vi "MQTT Packet - Receive.vi"(0 "mqtt ref in":T1, 7 "timeout (global)":i32=-1, 11 "error in":errorcluster) -> (3 "RAW data":string, 4 "mqtt ref out":T1, 6 "Fixed Header":T2, 8 "Remaining Data":u8[](array[numeric]), 10 "TimedOut":bool, 15 "error out":errorcluster)   [LabVIEW 2019, in "KoRE-MQTT.lvlib"]
doc: "Copyright (c) 2025 KoRElibs.com\nSPDX-License-Identifier: EUPL-1.2\n\nThis VI is licensed under the European Union Public License (EUPL) Version 1.2. You may use this VI unmodified in proprietary works. If you distribute a modified version of this file, the modified file must be released under the EUPL-1.2. Full license: https://joinup.ec.europa.eu/asset/eupl/eupl/1.2/"
uses:
  KoRE-MQTT.lvlib
  TypeDefs/MQTT Packet - Fixed Header.ctl
  TypeDefs/MQTT Packet - Type.ctl
  Public/TypeDefs/MQTT Client Session.ctl
  MQTT Data Stream - Decode Varint.vi
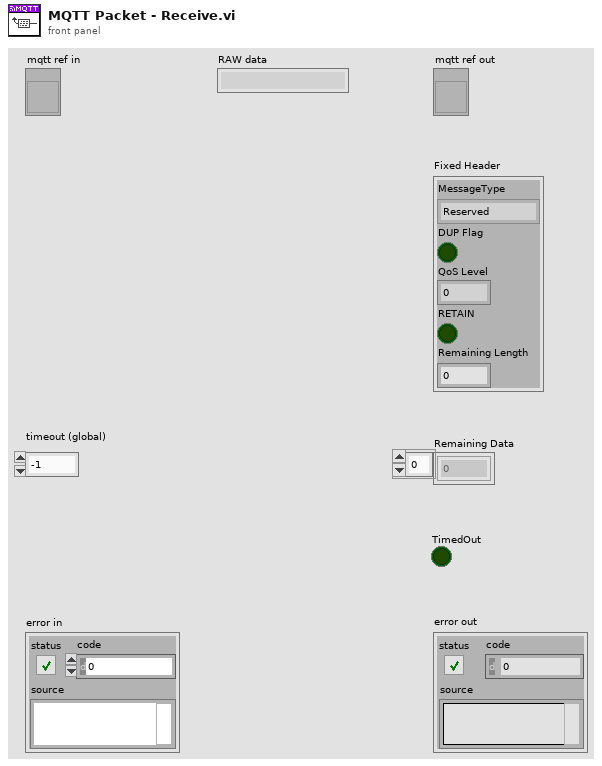
[diagram p1: front panel]
types:
  T1 = typedef "KoRE-MQTT.lvlib/MQTT Client Session.ctl" = refnum<vi>
  T2 = typedef "KoRE-MQTT.lvlib/MQTT Packet - Fixed Header.ctl" = cluster{"MessageType":T3, "DUP Flag":bool, "QoS Level":u8, "RETAIN":bool, "Remaining Length":u32}
  T3 = typedef "KoRE-MQTT.lvlib/MQTT Packet - Type.ctl" = enum32{"Reserved", "CONNECT", "CONNACK", "PUBLISH", "PUBACK", "PUBREC", "PUBREL", "PUBCOMP", "SUBSCRIBE", "SUBACK", "UNSUBSCRIBE", "UNSUBACK", "PINGREQ", "PINGRESP", "DISCONNECT", "AUTH"}
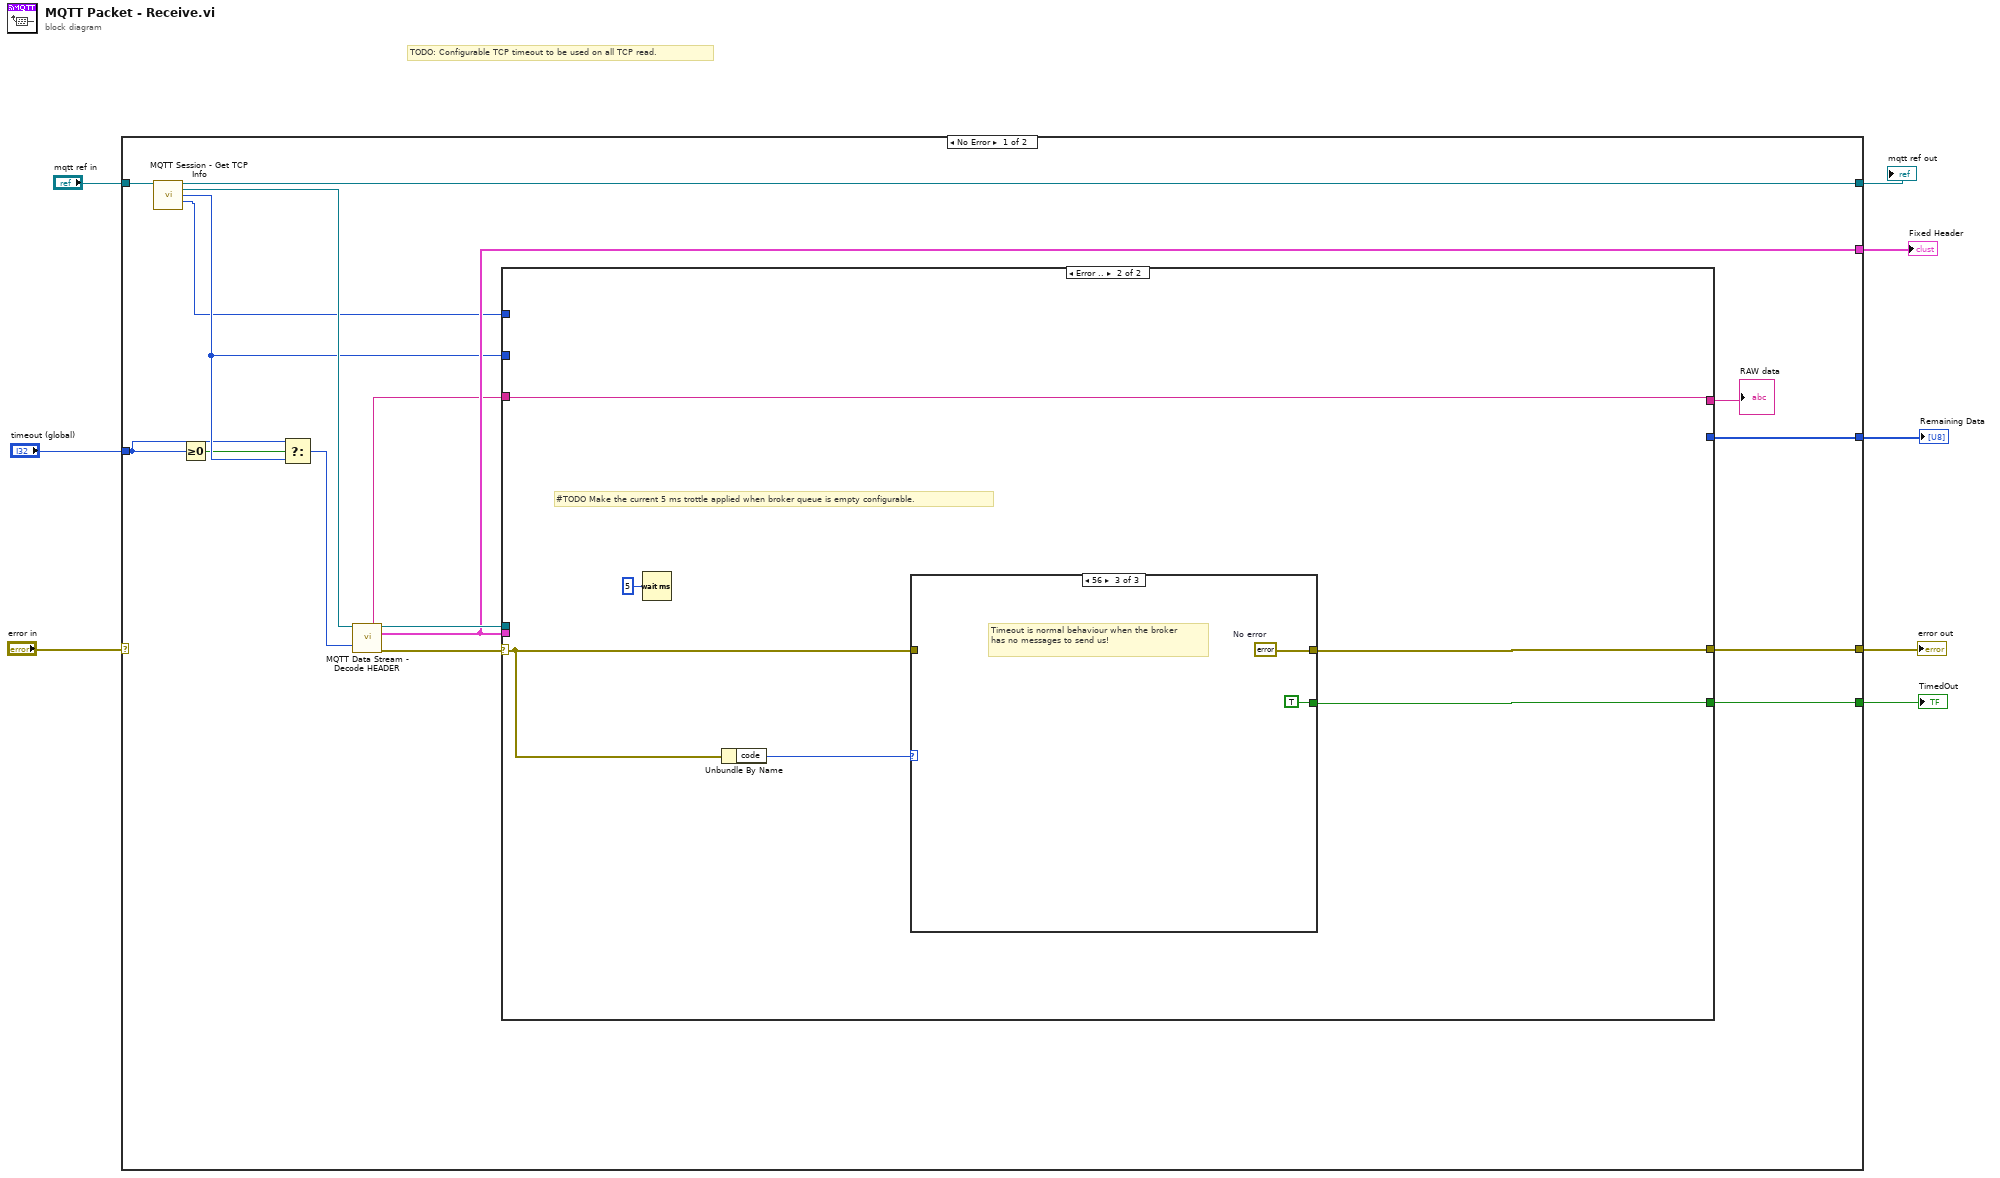
[diagram p0: block diagram]
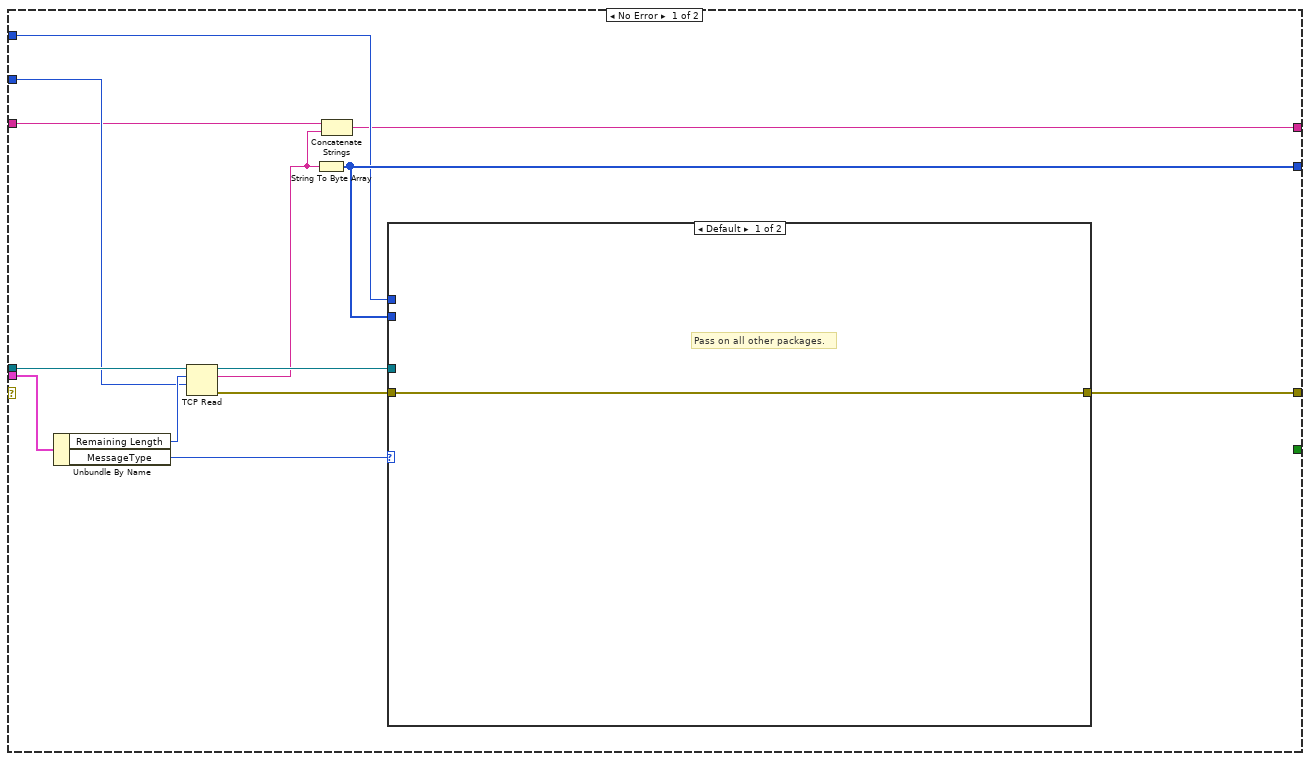
[diagram p2: hidden frame]
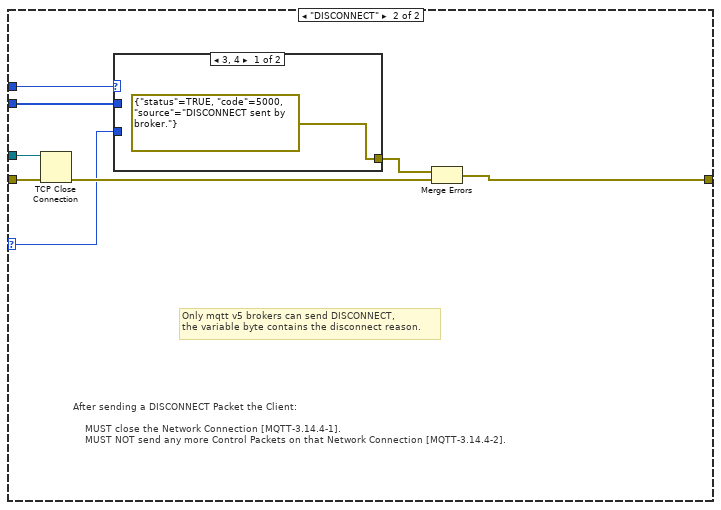
[diagram p3: hidden frame]
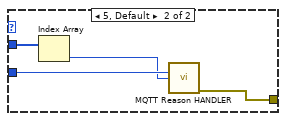
[diagram p4: hidden frame]
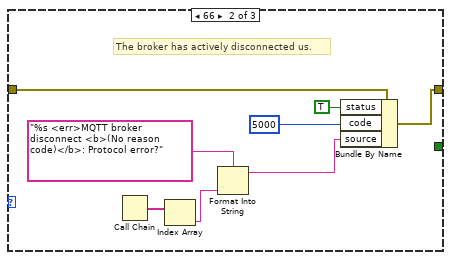
[diagram p6: hidden frame]
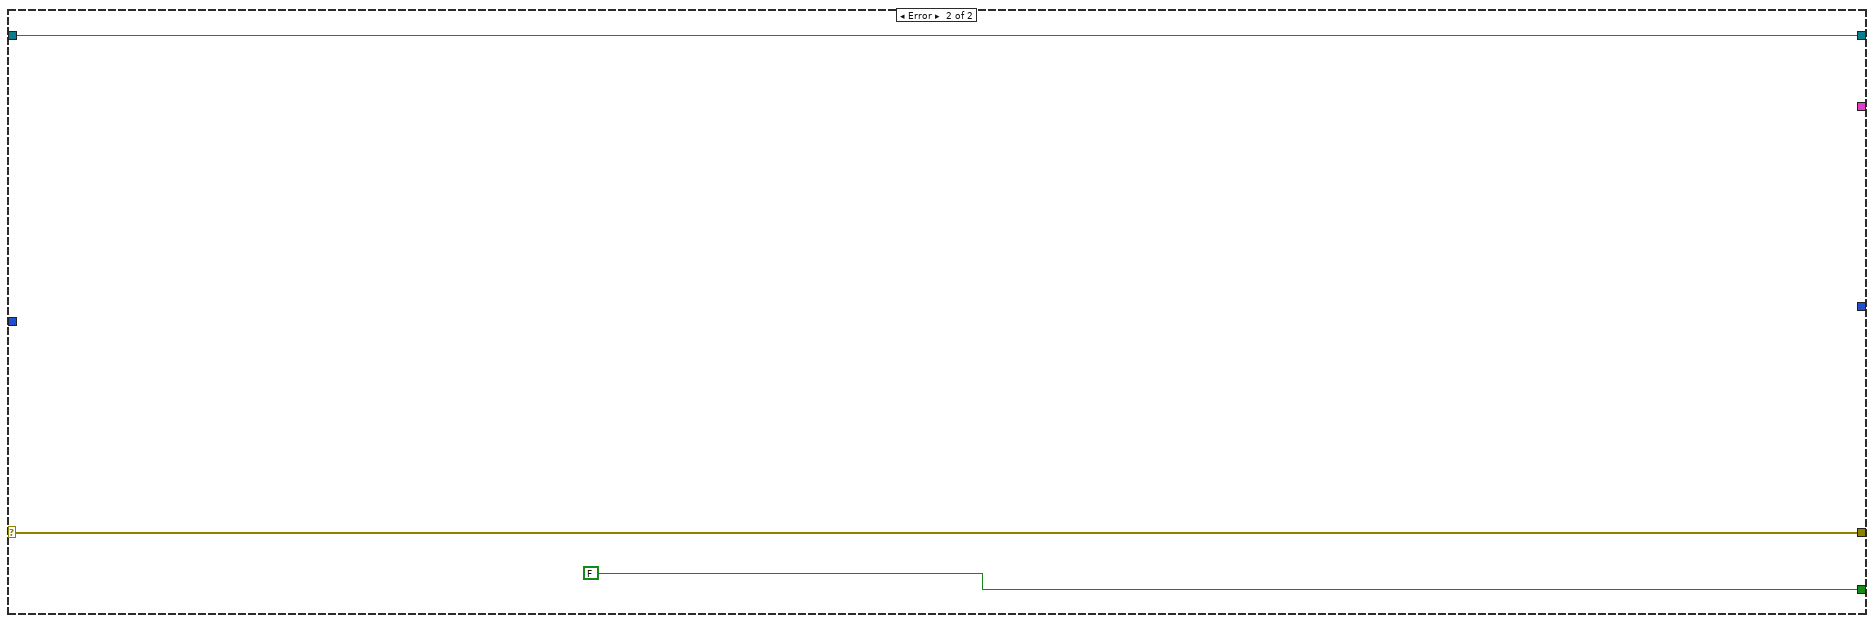
[diagram p7: hidden frame]
diagram:
  # "TODO: Configurable TCP timeout to be used on all TCP read."
  n1 = case shown="No Error" "error in" {
    selector: "error in" -> [_ w69]
    tunnel: [w15 w69] -> w8
    tunnel: [w14 FALSE] -> w6
    tunnel: [w23 _] -> w5
    tunnel: [w22 _] -> w4
    tunnel: "mqtt ref in" -> [w19 w70]
    tunnel: [w18 w70] -> w2
    tunnel: "timeout (global)" -> [w9 _]
    frame No Error {
      n2 = call "MQTT Session - Get TCP Info.vi"("mqtt ref in"=w19) -> ("mqtt ref out"=w18:T1, "TCP ref"=w17:refnum<k5>, "TCP Timeout (ms)"=w16:i32, "Version"=w12:u8)  [unwired: 10 in, 1 out]
      n3 = Greater Or Equal To 0?(x=w9) -> (x >= 0?=w13:bool)
      n4 = Select(t=w9, s=w13, f=w16) -> (s? t:f=w21:i32)
      n5 = call "MQTT Data Stream - Decode HEADER.vi"("TCP ref"=w17, "timeout ms (1000)"=w21) -> ("RAW Data"=w11:string, "TCP ref out"=w24:refnum<k5>, "Fixed Header"=w23:T2, "error out"=w20:errorcluster)  [unwired: 10 in]
      n6 = case shown="Error .." w20 {
        selector: w20 -> [_ w57]
        tunnel: [w30 w55] -> w15
        tunnel: w24 -> [w37 _]
        tunnel: w23 -> [w34 _]
        tunnel: [w32 _] -> w22
        tunnel: w16 -> [w29 _]
        tunnel: [_ w54] -> w14
        tunnel: w12 -> [w28 _]
        tunnel: w11 -> [w27 w53]
        tunnel: [w25 w53] -> w10
        frame No Error {
          n7 = Unbundle By Name(w34) -> ("Remaining Length"=w33:u32, "MessageType"=w31:T3)
          n8 = TCP Read(connection ID=w37, bytes to read=w33, 9:w29) -> (connection ID out=w35:refnum<k5>, data out=w26:string, error out=w36:errorcluster)  [unwired: 2 in]
          n9 = String To Byte Array(string=w26) -> (unsigned byte array=w32:u8[])
          n10 = Concatenate Strings(w27, w26) -> (w25:string)
          n11 = case shown="Default" w31 {
            selector: w31 -> [_ w40]
            tunnel: w32 -> [_ w46]
            tunnel: w35 -> [_ w45]
            tunnel: w36 -> [w38 w44]
            tunnel: [w38 w43] -> w30
            tunnel: w28 -> [_ w41]
            frame Default {
              # "Pass on all other packages."
            }
            frame "DISCONNECT" {
              # "After sending a DISCONNECT Packet the Client:\n\n    MUST close the Network Connection [MQTT-3.14.4-1].\n    MUST NOT send any more Control Packets on that Network Connection [MQTT-3.14.4-2]."
              # "Only mqtt v5 brokers can send DISCONNECT,\nthe variable byte contains the disconnect reason."
              n12 = TCP Close Connection(connection ID=w45, error in (no error)=w44) -> (error out=w42:errorcluster)  [unwired: 1 in, 1 out]
              n13 = case shown="3, 4" w41 {
                tunnel: w46 -> [_ w51]
                tunnel: w40 -> [_ w50]
                tunnel: [errorcluster {"status"=TRUE, "code"=5000, "source"="DISCONNECT sent by broker."} ("error out") w48] -> w39
                frame 3, 4 {
                }
                frame 5, Default {
                  n14 = Index Array(array=w51) -> (element=w49:u8)  [unwired: 1 in]
                  n15 = call "MQTT Reason HANDLER.vi"("MessageType"=w50, "Reason Code"=w49) -> ("error out"=w48:errorcluster)  [unwired: 13 in]
                }
              }
              n16 = Merge Errors(w39, w42) -> (w43:errorcluster)
            }
          }
        }
        frame Error {
          # "#TODO Make the current 5 ms trottle applied when broker queue is empty configurable."
          n17 = Wait (ms)(milliseconds to wait=u32 5) -> ()  [unwired: 1 out]
          n18 = Unbundle By Name(w57) -> ("code"=w56:i32)
          n19 = case shown="56" w56 {
            tunnel: w57 -> [w58 w62 _]
            tunnel: [w58 w63 w67] -> w55
            tunnel: [_ _ TRUE] -> w54
            frame Default {
            }
            frame 66 {
              # "The broker has actively disconnected us."
              n20 = Call Chain() -> (call chain=w60:string[])
              n21 = Index Array(array=w60) -> (element=w59:string)  [unwired: 1 in]
              n22 = Format Into String(format string="%s <err>MQTT broker disconnect <b>(No reason code)</b>: Protocol error?", w59) -> (resulting string=w64:string)  [unwired: 2 in, 1 out]
              n23 = Bundle By Name(cluster=w62, "status"=TRUE, "code"=5000, "source"=w64) -> (w63:errorcluster)
            }
            frame 56 {
              w67 = errorcluster {"status"=FALSE, "code"=0, "source"=""}  # No error
              # "Timeout is normal behaviour when the broker has no messages to send us!"
            }
          }
        }
      }
      "RAW data" <- w10
    }
    frame Error {
    }
  }
  "error out" <- w8
  "TimedOut" <- w6
  "Fixed Header" <- w5
  "Remaining Data" <- w4
  "mqtt ref out" <- w2
